vi "UpravljanjeHidraulicnomPumpom.vi"() -> ()   [LabVIEW 2014]
uses:
  Control 1.ctl
  <vilib>/functionblocks/Edge Detection/Edge Detect/Edge Detect.vi
  <vilib>/functionblocks/FB Core/FB Core.xnode
  <vilib>/functionblocks/NI_FunctionBlock Libraries.lvlib
panel:
  in  "stop":bool
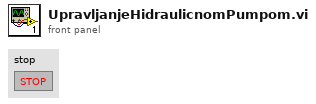
[diagram p1: front panel]
types:
  T1 = typedef "Control 1.ctl" = enum16{"System off", "System on", "Left", "Center", "Right", "Emergency off", ""}
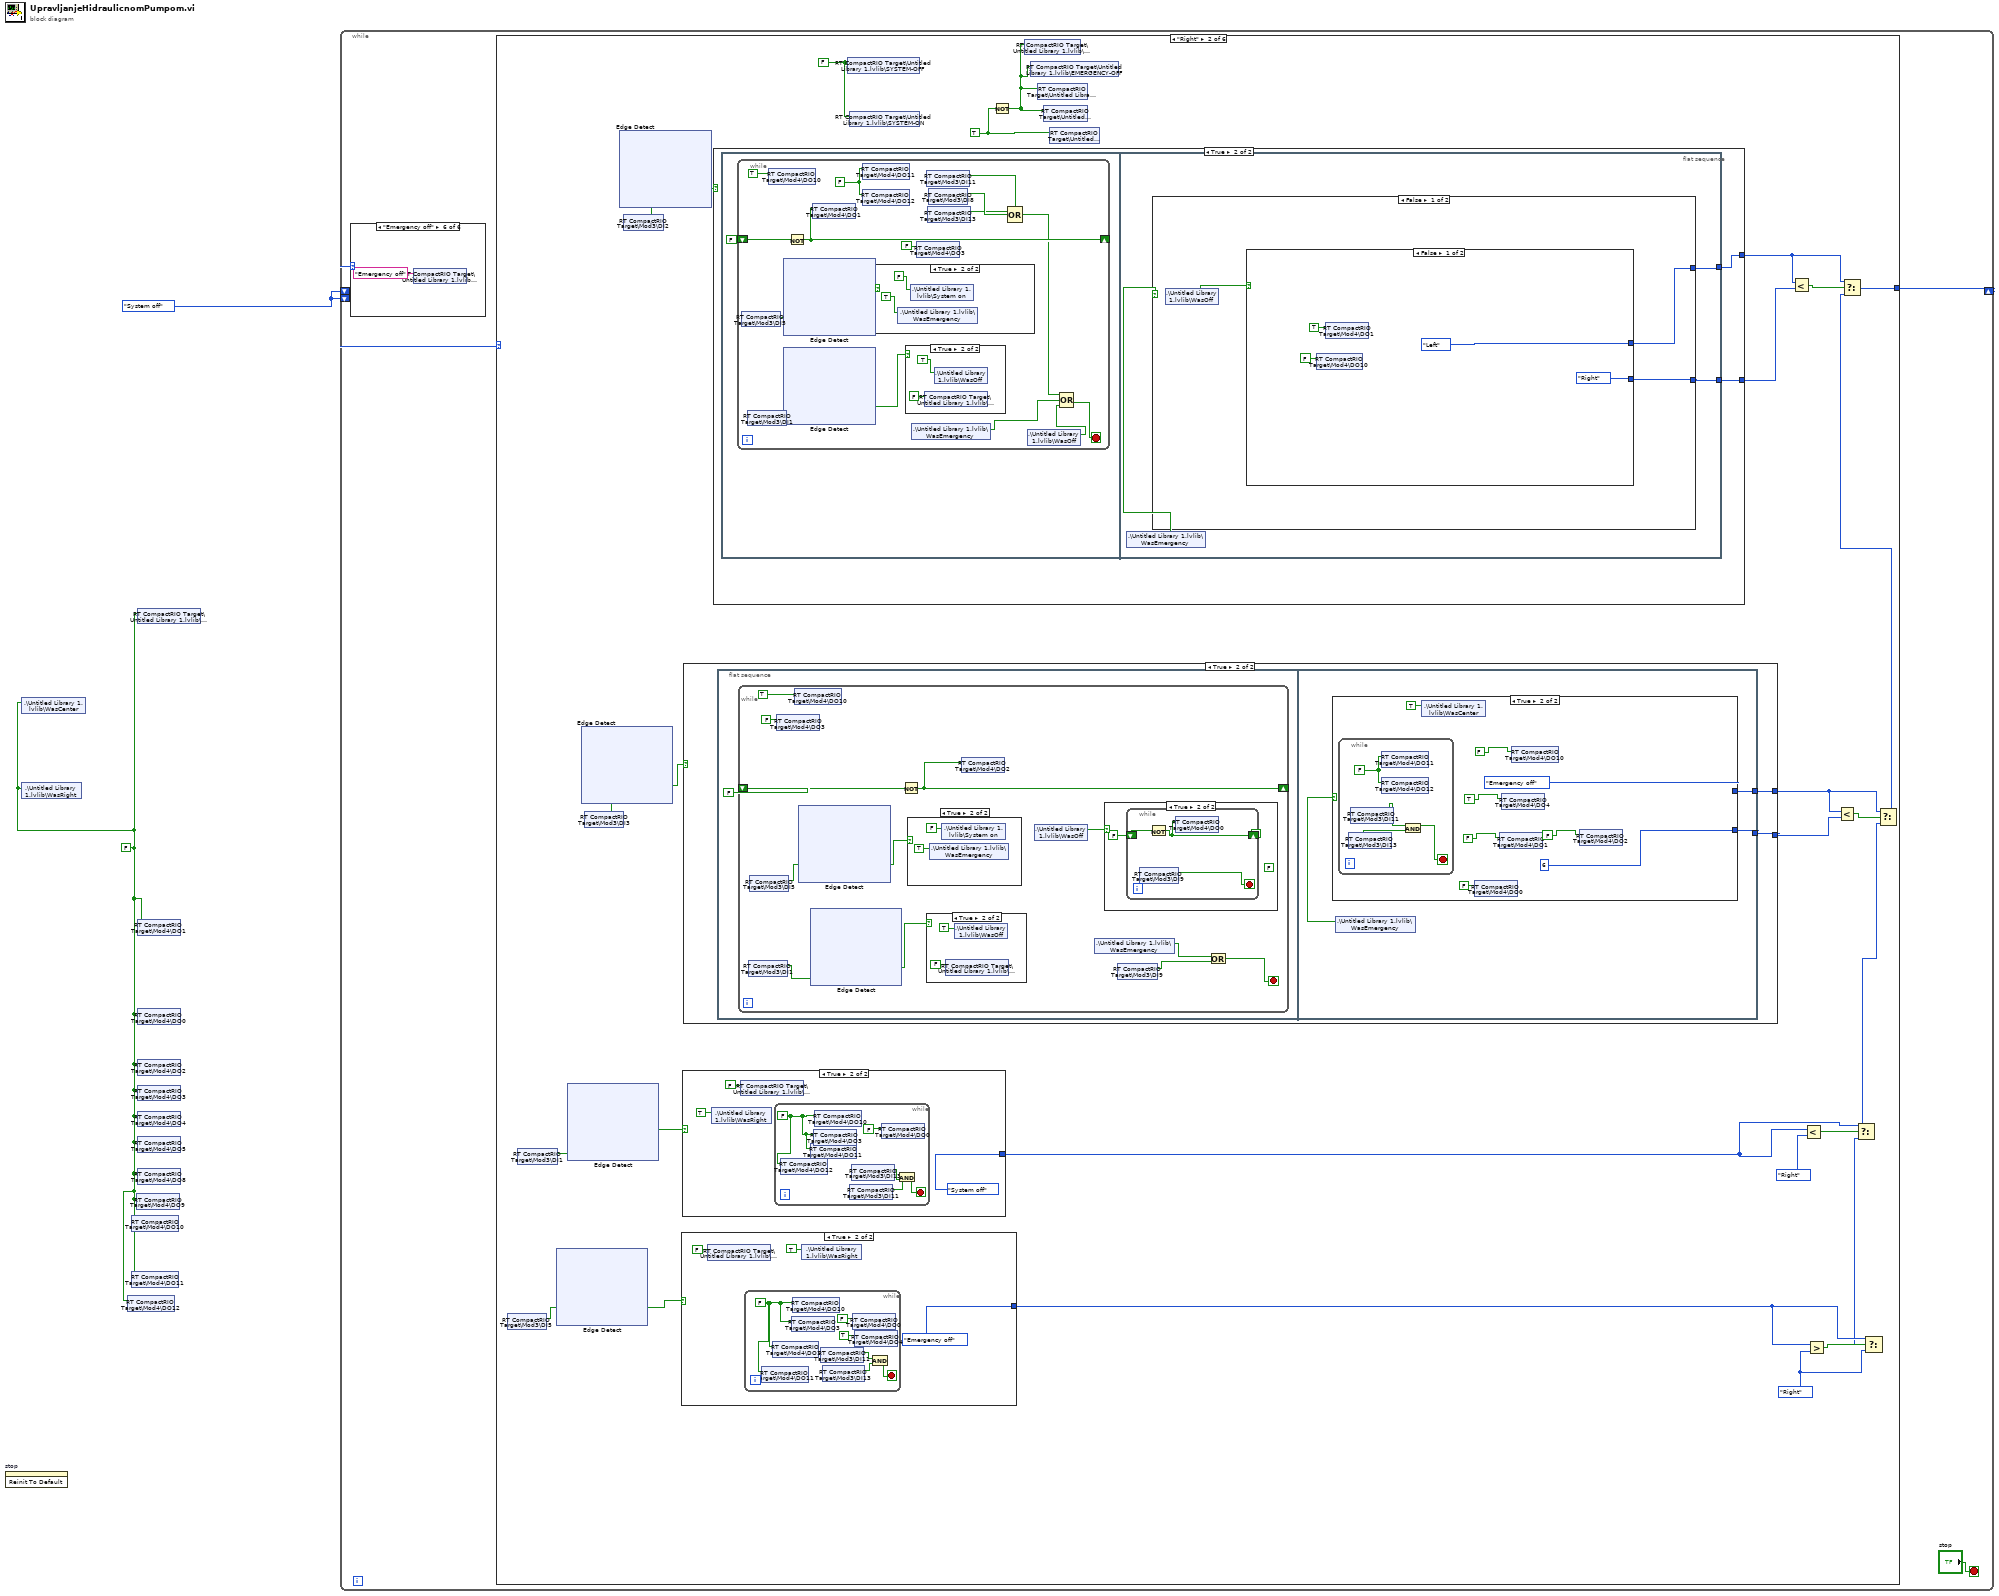
[diagram p0: block diagram]
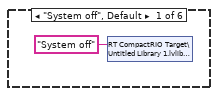
[diagram p2: hidden frame]
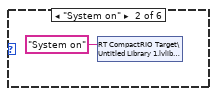
[diagram p3: hidden frame]
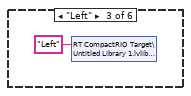
[diagram p4: hidden frame]
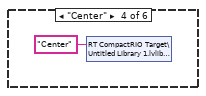
[diagram p5: hidden frame]
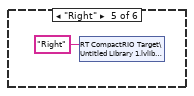
[diagram p6: hidden frame]
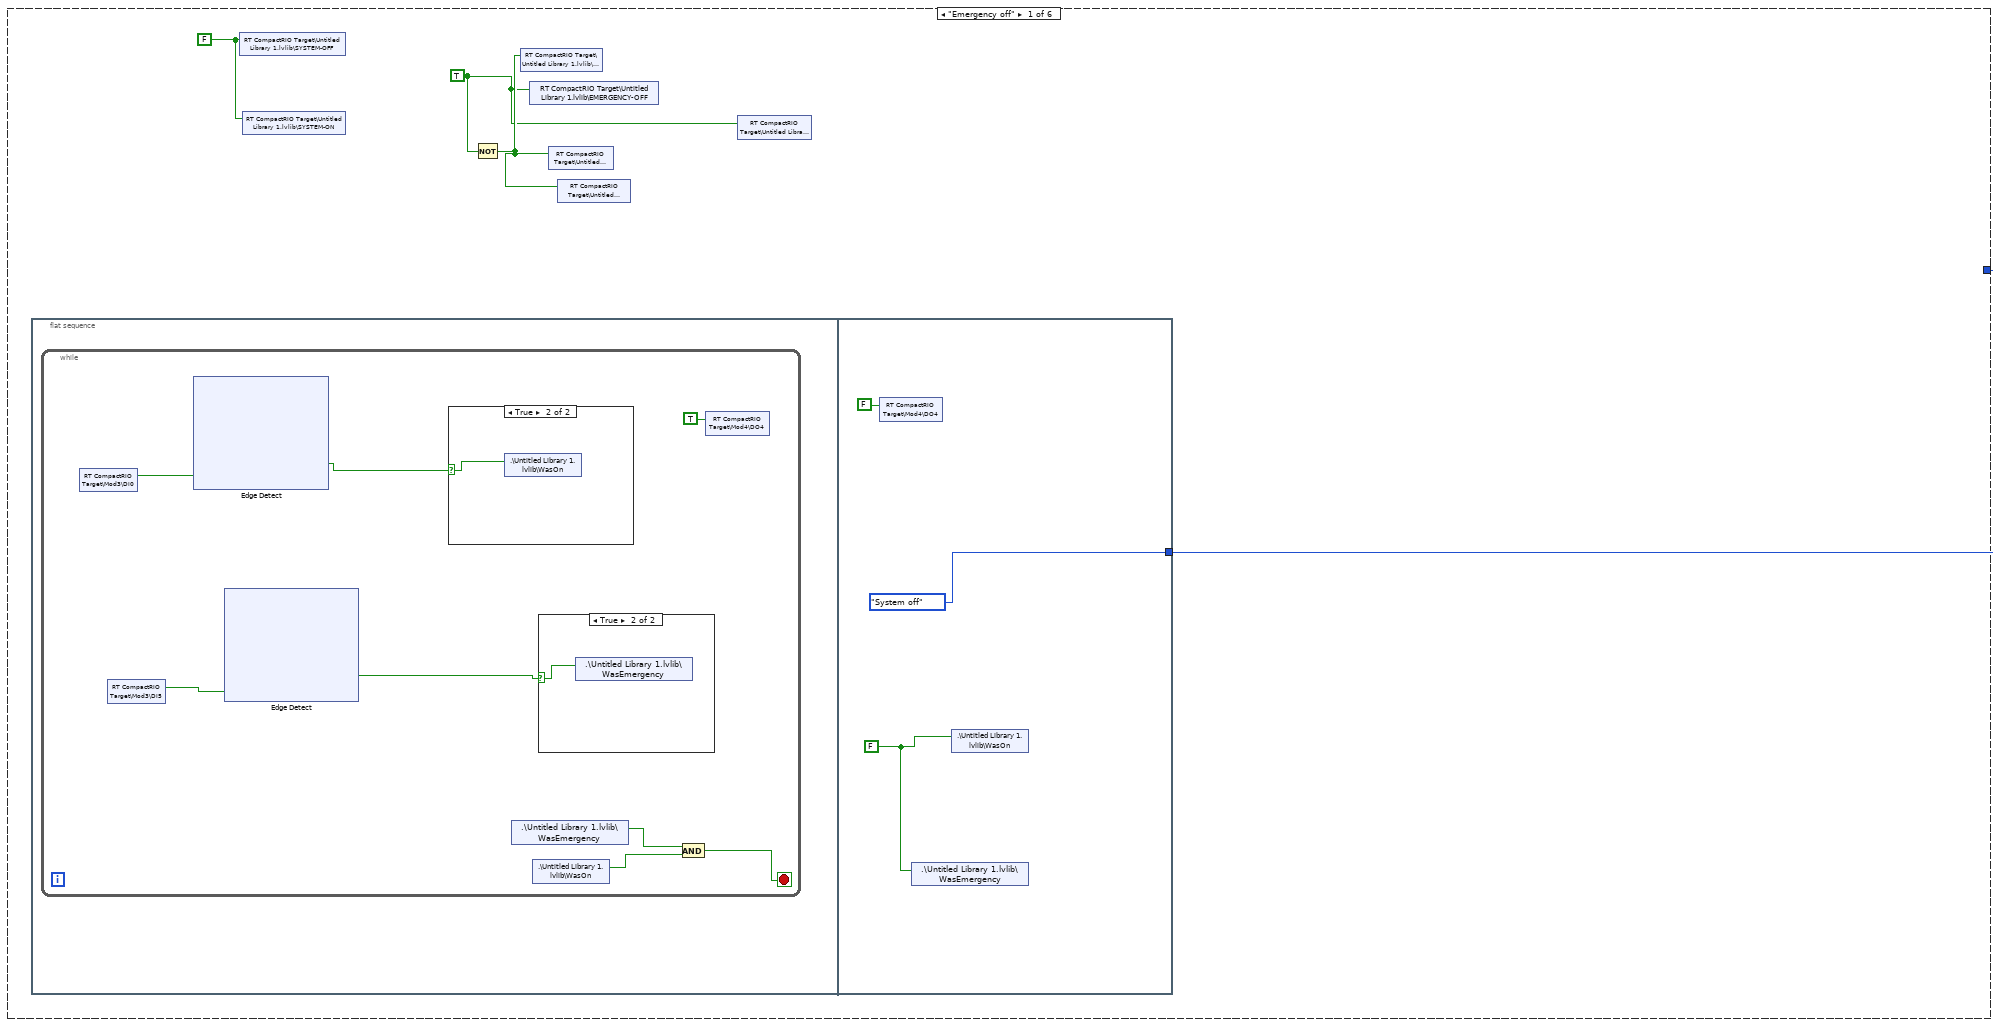
[diagram p7: hidden frame]
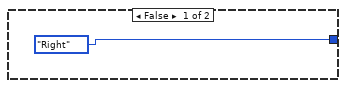
[diagram p10: hidden frame]
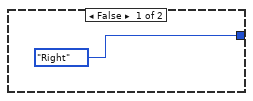
[diagram p11: hidden frame]
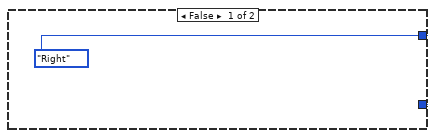
[diagram p12: hidden frame]
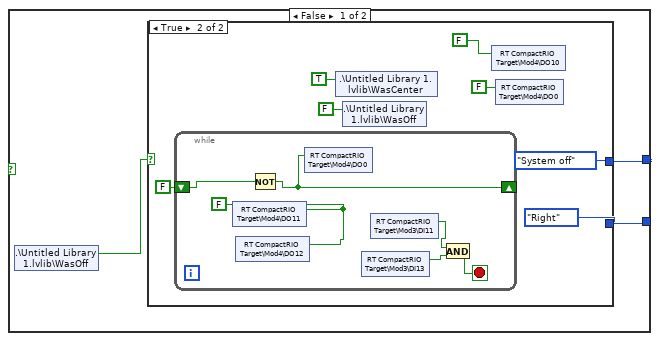
[diagram p16: hidden frame]
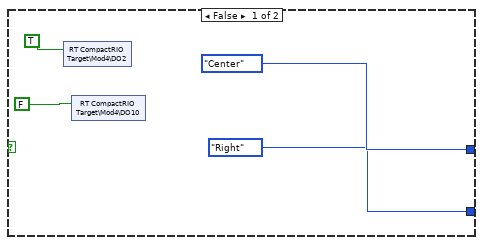
[diagram p17: hidden frame]
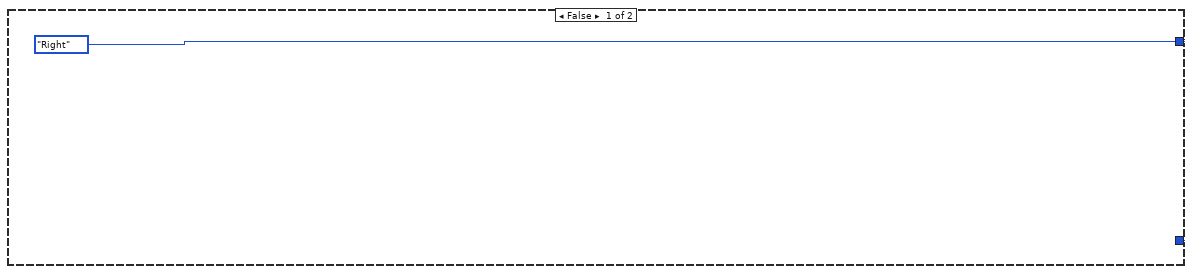
[diagram p18: hidden frame]
diagram:
  w2 = Control_1."System off" ("Enum")
  w1 = FALSE ("System on")
  n1 = invoke on="stop" class="Bool (strict)" method="Reinit To Default"() -> ()  [unwired: 3 in, 3 out]
  n2 = shared-variable ".\\Untitled Library 1.lvlib\\WasCenter"(w1) -> ()  [unwired: 1 in, 1 out]
  n3 = shared-variable ".\\Untitled Library 1.lvlib\\WasRight"(w1) -> ()  [unwired: 1 in, 1 out]
  n4 = shared-variable "RT CompactRIO Target\\Mod4\\DO12"(w1) -> ()  [unwired: 1 in, 1 out]
  n5 = shared-variable "RT CompactRIO Target\\Mod4\\DO10"(w1) -> ()  [unwired: 1 in, 1 out]
  n6 = shared-variable "RT CompactRIO Target\\Mod4\\DO11"(w1) -> ()  [unwired: 1 in, 1 out]
  n7 = shared-variable "RT CompactRIO Target\\Mod4\\DO9"(w1) -> ()  [unwired: 1 in, 1 out]
  n8 = shared-variable "RT CompactRIO Target\\Untitled Library 1.lvlib\\System on"(w1) -> ()  [unwired: 1 in, 1 out]
  n9 = shared-variable "RT CompactRIO Target\\Mod4\\DO1"(w1) -> ()  [unwired: 1 in, 1 out]
  n10 = shared-variable "RT CompactRIO Target\\Mod4\\DO0"(w1) -> ()  [unwired: 1 in, 1 out]
  n11 = shared-variable "RT CompactRIO Target\\Mod4\\DO2"(w1) -> ()  [unwired: 1 in, 1 out]
  n12 = shared-variable "RT CompactRIO Target\\Mod4\\DO3"(w1) -> ()  [unwired: 1 in, 1 out]
  n13 = shared-variable "RT CompactRIO Target\\Mod4\\DO4"(w1) -> ()  [unwired: 1 in, 1 out]
  n14 = shared-variable "RT CompactRIO Target\\Mod4\\DO5"(w1) -> ()  [unwired: 1 in, 1 out]
  n15 = shared-variable "RT CompactRIO Target\\Mod4\\DO8"(w1) -> ()  [unwired: 1 in, 1 out]
  n16 = while {
    shift-right: [w4] -> _
    shift-left: w2 -> [w3]
    shift-left: w2 -> [_]
    stop <- "stop" stop-if-true
    n17 = case shown="\"Emergency off\"" w3 {
      frame "System off", Default {
        n18 = shared-variable "RT CompactRIO Target\\Untitled Library 1.lvlib\\STANJE"("System off" ("STANJE")) -> ()  [unwired: 1 in, 1 out]
      }
      frame "System on" {
        n19 = shared-variable "RT CompactRIO Target\\Untitled Library 1.lvlib\\STANJE"("System on" ("STANJE")) -> ()  [unwired: 1 in, 1 out]
      }
      frame "Left" {
        n20 = shared-variable "RT CompactRIO Target\\Untitled Library 1.lvlib\\STANJE"("Left" ("STANJE")) -> ()  [unwired: 1 in, 1 out]
      }
      frame "Center" {
        n21 = shared-variable "RT CompactRIO Target\\Untitled Library 1.lvlib\\STANJE"("Center" ("STANJE")) -> ()  [unwired: 1 in, 1 out]
      }
      frame "Right" {
        n22 = shared-variable "RT CompactRIO Target\\Untitled Library 1.lvlib\\STANJE"("Right" ("STANJE")) -> ()  [unwired: 1 in, 1 out]
      }
      frame "Emergency off" {
        n23 = shared-variable "RT CompactRIO Target\\Untitled Library 1.lvlib\\STANJE"("Emergency off" ("STANJE")) -> ()  [unwired: 1 in, 1 out]
      }
    }
    n24 = case shown="\"Right\"" w3 {
      tunnel: [w15 w110 w592 w1059 w1532 w1594] -> w4
      frame "Emergency off" {
        w13 = FALSE ("SYSTEM-OFF")
        w12 = TRUE ("RIGHT")
        n25 = flat-sequence {
          tunnel: [Control_1."System off" ("Enum")] -> w15
          frame #0 {
            n26 = while {
              stop <- w21 stop-if-true
              n27 = shared-variable "RT CompactRIO Target\\Mod3\\DI0"() -> (w19:bool)  [unwired: 1 in, 1 out]
              n28 = shared-variable "RT CompactRIO Target\\Mod3\\DI5"() -> (w18:bool)  [unwired: 1 in, 1 out]
              n29 = xnode "Edge Detect"("input 1"=w19) -> ("output"=w17:bool)  [unwired: 2 in, 1 out]
              n30 = xnode "Edge Detect"("input 1"=w18) -> ("output"=w16:bool)  [unwired: 2 in, 1 out]
              n31 = case shown="True" w17 {
                selector: w17 -> [_ w25]
                frame False {
                }
                frame True {
                  n32 = shared-variable ".\\Untitled Library 1.lvlib\\WasOn"(w25) -> ()  [unwired: 1 in, 1 out]
                }
              }
              n33 = shared-variable ".\\Untitled Library 1.lvlib\\WasEmergency"() -> (w22:bool)  [unwired: 1 in, 1 out]
              n34 = shared-variable ".\\Untitled Library 1.lvlib\\WasOn"() -> (w23:bool)  [unwired: 1 in, 1 out]
              n35 = case shown="True" w16 {
                selector: w16 -> [_ w24]
                frame False {
                }
                frame True {
                  n36 = shared-variable ".\\Untitled Library 1.lvlib\\WasEmergency"(w24) -> ()  [unwired: 1 in, 1 out]
                }
              }
              n37 = And(x=w22, y=w23) -> (x .and. y?=w21:bool)
              n38 = shared-variable "RT CompactRIO Target\\Mod4\\DO4"(TRUE ("DO4")) -> ()  [unwired: 1 in, 1 out]
            }
          }
          frame #1 {
            w106 = FALSE ("WasOn")
            n39 = shared-variable "RT CompactRIO Target\\Mod4\\DO4"(FALSE ("DO4")) -> ()  [unwired: 1 in, 1 out]
            n40 = shared-variable ".\\Untitled Library 1.lvlib\\WasEmergency"(w106) -> ()  [unwired: 1 in, 1 out]
            n41 = shared-variable ".\\Untitled Library 1.lvlib\\WasOn"(w106) -> ()  [unwired: 1 in, 1 out]
          }
        }
        n42 = shared-variable "RT CompactRIO Target\\Untitled Library 1.lvlib\\SYSTEM-OFF"(w13) -> ()  [unwired: 1 in, 1 out]
        n43 = shared-variable "RT CompactRIO Target\\Untitled Library 1.lvlib\\SYSTEM-ON"(w13) -> ()  [unwired: 1 in, 1 out]
        n44 = Not(x=w12) -> (.not. x?=w14:bool)
        n45 = shared-variable "RT CompactRIO Target\\Untitled Library 1.lvlib\\CENTER"(w14) -> ()  [unwired: 1 in, 1 out]
        n46 = shared-variable "RT CompactRIO Target\\Untitled Library 1.lvlib\\EMERGENCY-OFF"(w12) -> ()  [unwired: 1 in, 1 out]
        n47 = shared-variable "RT CompactRIO Target\\Untitled Library 1.lvlib\\LEFT"(w14) -> ()  [unwired: 1 in, 1 out]
        n48 = shared-variable "RT CompactRIO Target\\Untitled Library 1.lvlib\\RIGHT"(w14) -> ()  [unwired: 1 in, 1 out]
        n49 = shared-variable "RT CompactRIO Target\\Untitled Library 1.lvlib\\FAULT"(w12) -> ()  [unwired: 1 in, 1 out]
      }
      frame "Right" {
        w109 = FALSE ("SYSTEM-OFF")
        w111 = Control_1."Right" ("y")
        w127 = TRUE ("RIGHT")
        n50 = shared-variable "RT CompactRIO Target\\Mod3\\DI5"() -> (w128:bool)  [unwired: 1 in, 1 out]
        n51 = shared-variable "RT CompactRIO Target\\Mod3\\DI1"() -> (w129:bool)  [unwired: 1 in, 1 out]
        n52 = xnode "Edge Detect"("input 2"=w128) -> ("output"=w130:bool)  [unwired: 2 in, 1 out]
        n53 = xnode "Edge Detect"("input 1"=w129) -> ("output"=w131:bool)  [unwired: 2 in, 1 out]
        n54 = shared-variable "RT CompactRIO Target\\Mod3\\DI3"() -> (w133:bool)  [unwired: 1 in, 1 out]
        n55 = xnode "Edge Detect"("input 1"=w133) -> ("output"=w132:bool)  [unwired: 2 in, 1 out]
        n56 = shared-variable "RT CompactRIO Target\\Mod3\\DI2"() -> (w135:bool)  [unwired: 1 in, 1 out]
        n57 = xnode "Edge Detect"("input 1"=w135) -> ("output"=w134:bool)  [unwired: 2 in, 1 out]
        n58 = case shown="True" w130 {
          tunnel: [Control_1."Right" ("Enum") Control_1."Emergency off" ("Enum")] -> w113
          frame False {
          }
          frame True {
            n59 = shared-variable "RT CompactRIO Target\\Untitled Library 1.lvlib\\System on"(FALSE ("System on")) -> ()  [unwired: 1 in, 1 out]
            n60 = while {
              stop <- w143 stop-if-true
              w142 = FALSE ("DO8")
              n61 = shared-variable "RT CompactRIO Target\\Mod4\\DO11"(w142) -> ()  [unwired: 1 in, 1 out]
              n62 = shared-variable "RT CompactRIO Target\\Mod4\\DO12"(w142) -> ()  [unwired: 1 in, 1 out]
              n63 = shared-variable "RT CompactRIO Target\\Mod4\\DO3"(w142) -> ()  [unwired: 1 in, 1 out]
              n64 = shared-variable "RT CompactRIO Target\\Mod4\\DO10"(w142) -> ()  [unwired: 1 in, 1 out]
              n65 = shared-variable "RT CompactRIO Target\\Mod3\\DI11"() -> (w144:bool)  [unwired: 1 in, 1 out]
              n66 = shared-variable "RT CompactRIO Target\\Mod3\\DI13"() -> (w145:bool)  [unwired: 1 in, 1 out]
              n67 = shared-variable "RT CompactRIO Target\\Mod4\\DO0"(FALSE ("DO4")) -> ()  [unwired: 1 in, 1 out]
              n68 = shared-variable "RT CompactRIO Target\\Mod4\\DO4"(TRUE ("DO4")) -> ()  [unwired: 1 in, 1 out]
              n69 = And(x=w144, y=w145) -> (x .and. y?=w143:bool)
            }
            n70 = shared-variable ".\\Untitled Library 1.lvlib\\WasRight"(TRUE ("WasCenter")) -> ()  [unwired: 1 in, 1 out]
          }
        }
        n71 = case shown="True" w131 {
          tunnel: [Control_1."Right" ("Enum") Control_1."System off" ("Enum")] -> w116
          frame False {
          }
          frame True {
            n72 = shared-variable ".\\Untitled Library 1.lvlib\\WasRight"(TRUE ("WasCenter")) -> ()  [unwired: 1 in, 1 out]
            n73 = shared-variable "RT CompactRIO Target\\Untitled Library 1.lvlib\\System on"(FALSE ("System on")) -> ()  [unwired: 1 in, 1 out]
            n74 = while {
              stop <- w192 stop-if-true
              w191 = FALSE ("DO8")
              n75 = shared-variable "RT CompactRIO Target\\Mod4\\DO12"(w191) -> ()  [unwired: 1 in, 1 out]
              n76 = shared-variable "RT CompactRIO Target\\Mod4\\DO11"(w191) -> ()  [unwired: 1 in, 1 out]
              n77 = shared-variable "RT CompactRIO Target\\Mod4\\DO3"(w191) -> ()  [unwired: 1 in, 1 out]
              n78 = shared-variable "RT CompactRIO Target\\Mod4\\DO10"(w191) -> ()  [unwired: 1 in, 1 out]
              n79 = shared-variable "RT CompactRIO Target\\Mod3\\DI11"() -> (w193:bool)  [unwired: 1 in, 1 out]
              n80 = shared-variable "RT CompactRIO Target\\Mod3\\DI13"() -> (w194:bool)  [unwired: 1 in, 1 out]
              n81 = shared-variable "RT CompactRIO Target\\Mod4\\DO0"(FALSE ("DO8")) -> ()  [unwired: 1 in, 1 out]
              n82 = And(x=w193, y=w194) -> (x .and. y?=w192:bool)
            }
          }
        }
        n83 = case shown="True" w132 {
          tunnel: [w235 w237] -> w120
          tunnel: [w235 w236] -> w122
          frame False {
            w235 = Control_1."Right" ("Enum")
          }
          frame True {
            n84 = flat-sequence {
              tunnel: [w340] -> w237
              tunnel: [w339] -> w236
              frame #0 {
                n85 = while {
                  shift-right: [w249] -> _
                  shift-left: FALSE ("DO8") -> [w250]
                  stop <- w242 stop-if-true
                  n86 = shared-variable "RT CompactRIO Target\\Mod3\\DI1"() -> (w240:bool)  [unwired: 1 in, 1 out]
                  n87 = shared-variable "RT CompactRIO Target\\Mod3\\DI5"() -> (w246:bool)  [unwired: 1 in, 1 out]
                  n88 = shared-variable "RT CompactRIO Target\\Mod4\\DO3"(FALSE ("DO3")) -> ()  [unwired: 1 in, 1 out]
                  n89 = shared-variable "RT CompactRIO Target\\Mod4\\DO10"(TRUE ("DO8")) -> ()  [unwired: 1 in, 1 out]
                  n90 = xnode "Edge Detect"("input 2"=w246) -> ("output"=w245:bool)  [unwired: 2 in, 1 out]
                  n91 = xnode "Edge Detect"("input 1"=w240) -> ("output"=w239:bool)  [unwired: 2 in, 1 out]
                  n92 = Not(x=w250) -> (.not. x?=w249:bool)
                  n93 = case shown="True" w245 {
                    frame False {
                    }
                    frame True {
                      n94 = shared-variable ".\\Untitled Library 1.lvlib\\WasEmergency"(TRUE ("WasEmergency")) -> ()  [unwired: 1 in, 1 out]
                      n95 = shared-variable ".\\Untitled Library 1.lvlib\\System on"(FALSE ("System on")) -> ()  [unwired: 1 in, 1 out]
                    }
                  }
                  n96 = case shown="True" w239 {
                    frame False {
                    }
                    frame True {
                      n97 = shared-variable "RT CompactRIO Target\\Untitled Library 1.lvlib\\System on"(FALSE ("System on")) -> ()  [unwired: 1 in, 1 out]
                      n98 = shared-variable ".\\Untitled Library 1.lvlib\\WasOff"(TRUE ("WasOff")) -> ()  [unwired: 1 in, 1 out]
                    }
                  }
                  n99 = shared-variable "RT CompactRIO Target\\Mod4\\DO2"(w249) -> ()  [unwired: 1 in, 1 out]
                  n100 = shared-variable ".\\Untitled Library 1.lvlib\\WasOff"() -> (w241:bool)  [unwired: 1 in, 1 out]
                  n101 = shared-variable ".\\Untitled Library 1.lvlib\\WasEmergency"() -> (w244:bool)  [unwired: 1 in, 1 out]
                  n102 = case shown="True" w241 {
                    frame False {
                    }
                    frame True {
                      (unwired) FALSE ("WasOff")
                      (unwired) FALSE ("DO8")
                      n103 = while {
                        shift-right: [w252] -> _
                        shift-left: FALSE -> [w254]
                        stop <- w253 stop-if-true
                        n104 = shared-variable "RT CompactRIO Target\\Mod3\\DI9"() -> (w253:bool)  [unwired: 1 in, 1 out]
                        n105 = Not(x=w254) -> (.not. x?=w252:bool)
                        n106 = shared-variable "RT CompactRIO Target\\Mod4\\DO0"(w252) -> ()  [unwired: 1 in, 1 out]
                      }
                    }
                  }
                  n107 = shared-variable "RT CompactRIO Target\\Mod3\\DI9"() -> (w243:bool)  [unwired: 1 in, 1 out]
                  n108 = Or(x=w244, y=w243) -> (x .or. y?=w242:bool)
                }
              }
              frame #1 {
                n109 = shared-variable ".\\Untitled Library 1.lvlib\\WasEmergency"() -> (w341:bool)  [unwired: 1 in, 1 out]
                n110 = case shown="True" w341 {
                  tunnel: [w343 Control_1."Emergency off" ("Enum")] -> w340
                  tunnel: [w342 6] -> w339
                  frame False {
                    n111 = shared-variable ".\\Untitled Library 1.lvlib\\WasOff"() -> (w344:bool)  [unwired: 1 in, 1 out]
                    n112 = case shown="True" w344 {
                      tunnel: [Control_1."Center" ("Enum") Control_1."System off" ("Enum")] -> w343
                      tunnel: [Control_1."Right" ("Enum") Control_1."Right" ("Enum")] -> w342
                      frame False {
                        n113 = shared-variable "RT CompactRIO Target\\Mod4\\DO2"(TRUE ("DO12")) -> ()  [unwired: 1 in, 1 out]
                        n114 = shared-variable "RT CompactRIO Target\\Mod4\\DO10"(FALSE ("DO8")) -> ()  [unwired: 1 in, 1 out]
                      }
                      frame True {
                        n115 = while {
                          shift-right: [w356] -> _
                          shift-left: FALSE -> [w357]
                          stop <- w358 stop-if-true
                          w361 = FALSE ("DO11")
                          n116 = shared-variable "RT CompactRIO Target\\Mod4\\DO11"(w361) -> ()  [unwired: 1 in, 1 out]
                          n117 = shared-variable "RT CompactRIO Target\\Mod4\\DO12"(w361) -> ()  [unwired: 1 in, 1 out]
                          n118 = Not(x=w357) -> (.not. x?=w356:bool)
                          n119 = shared-variable "RT CompactRIO Target\\Mod4\\DO0"(w356) -> ()  [unwired: 1 in, 1 out]
                          n120 = shared-variable "RT CompactRIO Target\\Mod3\\DI13"() -> (w359:bool)  [unwired: 1 in, 1 out]
                          n121 = shared-variable "RT CompactRIO Target\\Mod3\\DI11"() -> (w360:bool)  [unwired: 1 in, 1 out]
                          n122 = And(x=w360, y=w359) -> (x .and. y?=w358:bool)
                        }
                        n123 = shared-variable ".\\Untitled Library 1.lvlib\\WasCenter"(TRUE ("WasRight")) -> ()  [unwired: 1 in, 1 out]
                        n124 = shared-variable ".\\Untitled Library 1.lvlib\\WasOff"(FALSE ("WasOff")) -> ()  [unwired: 1 in, 1 out]
                        n125 = shared-variable "RT CompactRIO Target\\Mod4\\DO10"(FALSE ("DO0")) -> ()  [unwired: 1 in, 1 out]
                        n126 = shared-variable "RT CompactRIO Target\\Mod4\\DO0"(FALSE ("DO0")) -> ()  [unwired: 1 in, 1 out]
                      }
                    }
                  }
                  frame True {
                    n127 = while {
                      stop <- w370 stop-if-true
                      w373 = FALSE ("DO8")
                      n128 = shared-variable "RT CompactRIO Target\\Mod3\\DI13"() -> (w371:bool)  [unwired: 1 in, 1 out]
                      n129 = shared-variable "RT CompactRIO Target\\Mod3\\DI11"() -> (w372:bool)  [unwired: 1 in, 1 out]
                      n130 = shared-variable "RT CompactRIO Target\\Mod4\\DO11"(w373) -> ()  [unwired: 1 in, 1 out]
                      n131 = shared-variable "RT CompactRIO Target\\Mod4\\DO12"(w373) -> ()  [unwired: 1 in, 1 out]
                      n132 = And(x=w372, y=w371) -> (x .and. y?=w370:bool)
                    }
                    n133 = shared-variable ".\\Untitled Library 1.lvlib\\WasCenter"(TRUE ("WasRight")) -> ()  [unwired: 1 in, 1 out]
                    n134 = shared-variable "RT CompactRIO Target\\Mod4\\DO0"(FALSE ("DO0")) -> ()  [unwired: 1 in, 1 out]
                    n135 = shared-variable "RT CompactRIO Target\\Mod4\\DO1"(FALSE ("DO8")) -> ()  [unwired: 1 in, 1 out]
                    n136 = shared-variable "RT CompactRIO Target\\Mod4\\DO4"(TRUE ("DO8")) -> ()  [unwired: 1 in, 1 out]
                    n137 = shared-variable "RT CompactRIO Target\\Mod4\\DO10"(FALSE ("DO8")) -> ()  [unwired: 1 in, 1 out]
                    n138 = shared-variable "RT CompactRIO Target\\Mod4\\DO2"(FALSE ("DO8")) -> ()  [unwired: 1 in, 1 out]
                  }
                }
              }
            }
          }
        }
        n139 = case shown="True" w134 {
          tunnel: [w414 w416] -> w123
          tunnel: [w414 w415] -> w125
          frame False {
            w414 = Control_1."Right" ("Enum")
          }
          frame True {
            n140 = flat-sequence {
              tunnel: [w519] -> w416
              tunnel: [w518] -> w415
              frame #0 {
                n141 = while {
                  shift-right: [w431] -> _
                  shift-left: FALSE ("DO8") -> [w432]
                  stop <- w420 stop-if-true
                  w427 = FALSE ("DO8")
                  n142 = shared-variable "RT CompactRIO Target\\Mod3\\DI5"() -> (w424:bool)  [unwired: 1 in, 1 out]
                  n143 = shared-variable "RT CompactRIO Target\\Mod3\\DI1"() -> (w425:bool)  [unwired: 1 in, 1 out]
                  n144 = shared-variable "RT CompactRIO Target\\Mod4\\DO10"(TRUE ("DO8")) -> ()  [unwired: 1 in, 1 out]
                  n145 = xnode "Edge Detect"("input 2"=w424) -> ("output"=w423:bool)  [unwired: 2 in, 1 out]
                  n146 = xnode "Edge Detect"("input 1"=w425) -> ("output"=w419:bool)  [unwired: 2 in, 1 out]
                  n147 = Not(x=w432) -> (.not. x?=w431:bool)
                  n148 = shared-variable "RT CompactRIO Target\\Mod4\\DO1"(w431) -> ()  [unwired: 1 in, 1 out]
                  n149 = shared-variable "RT CompactRIO Target\\Mod4\\DO11"(w427) -> ()  [unwired: 1 in, 1 out]
                  n150 = shared-variable "RT CompactRIO Target\\Mod4\\DO12"(w427) -> ()  [unwired: 1 in, 1 out]
                  n151 = case shown="True" w423 {
                    frame False {
                    }
                    frame True {
                      n152 = shared-variable ".\\Untitled Library 1.lvlib\\WasEmergency"(TRUE ("WasEmergency")) -> ()  [unwired: 1 in, 1 out]
                      n153 = shared-variable ".\\Untitled Library 1.lvlib\\System on"(FALSE ("System on")) -> ()  [unwired: 1 in, 1 out]
                    }
                  }
                  n154 = case shown="True" w419 {
                    frame False {
                    }
                    frame True {
                      n155 = shared-variable "RT CompactRIO Target\\Untitled Library 1.lvlib\\System on"(FALSE ("System on")) -> ()  [unwired: 1 in, 1 out]
                      n156 = shared-variable ".\\Untitled Library 1.lvlib\\WasOff"(TRUE ("WasOff")) -> ()  [unwired: 1 in, 1 out]
                    }
                  }
                  n157 = shared-variable ".\\Untitled Library 1.lvlib\\WasEmergency"() -> (w421:bool)  [unwired: 1 in, 1 out]
                  n158 = shared-variable "RT CompactRIO Target\\Mod4\\DO3"(FALSE ("DO3")) -> ()  [unwired: 1 in, 1 out]
                  n159 = shared-variable "RT CompactRIO Target\\Mod3\\DI11"() -> (w430:bool)  [unwired: 1 in, 1 out]
                  n160 = shared-variable "RT CompactRIO Target\\Mod3\\DI13"() -> (w428:bool)  [unwired: 1 in, 1 out]
                  n161 = shared-variable "RT CompactRIO Target\\Mod3\\DI8"() -> (w429:bool)  [unwired: 1 in, 1 out]
                  n162 = Compound Arithmetic op=OR(w430, w429, w428) -> (w418:bool)
                  n163 = shared-variable ".\\Untitled Library 1.lvlib\\WasOff"() -> (w422:bool)  [unwired: 1 in, 1 out]
                  n164 = Compound Arithmetic op=OR(w418, w421, w422) -> (w420:bool)
                }
              }
              frame #1 {
                n165 = shared-variable ".\\Untitled Library 1.lvlib\\WasEmergency"() -> (w520:bool)  [unwired: 1 in, 1 out]
                n166 = case shown="False" w520 {
                  tunnel: [w522 Control_1."Emergency off" ("Enum")] -> w519
                  tunnel: [w521 6] -> w518
                  frame False {
                    n167 = shared-variable ".\\Untitled Library 1.lvlib\\WasOff"() -> (w523:bool)  [unwired: 1 in, 1 out]
                    n168 = case shown="False" w523 {
                      tunnel: [Control_1."Left" ("Enum") Control_1."System off" ("Enum")] -> w522
                      tunnel: [Control_1."Right" ("Enum") Control_1."Right" ("Enum")] -> w521
                      frame False {
                        n169 = shared-variable "RT CompactRIO Target\\Mod4\\DO10"(FALSE ("DO1")) -> ()  [unwired: 1 in, 1 out]
                        n170 = shared-variable "RT CompactRIO Target\\Mod4\\DO1"(TRUE ("DO3")) -> ()  [unwired: 1 in, 1 out]
                      }
                      frame True {
                        n171 = flat-sequence {
                          frame #0 {
                            n172 = while {
                              shift-right: [w538] -> _
                              shift-left: FALSE -> [w539]
                              stop <- w534 stop-if-true
                              w537 = FALSE ("DO8")
                              n173 = shared-variable "RT CompactRIO Target\\Mod4\\DO10"(TRUE ("DO1")) -> ()  [unwired: 1 in, 1 out]
                              n174 = shared-variable "RT CompactRIO Target\\Mod3\\DI13"() -> (w535:bool)  [unwired: 1 in, 1 out]
                              n175 = shared-variable "RT CompactRIO Target\\Mod3\\DI11"() -> (w536:bool)  [unwired: 1 in, 1 out]
                              n176 = shared-variable "RT CompactRIO Target\\Mod3\\DI8"() -> (w532:bool)  [unwired: 1 in, 1 out]
                              n177 = Not(x=w539) -> (.not. x?=w538:bool)
                              n178 = Compound Arithmetic op=AND(w536, w535, w532) -> (w534:bool)
                              n179 = shared-variable "RT CompactRIO Target\\Mod4\\DO11"(w537) -> ()  [unwired: 1 in, 1 out]
                              n180 = shared-variable "RT CompactRIO Target\\Mod4\\DO12"(w537) -> ()  [unwired: 1 in, 1 out]
                              n181 = shared-variable "RT CompactRIO Target\\Mod4\\DO0"(w538) -> ()  [unwired: 1 in, 1 out]
                            }
                          }
                          frame #1 {
                            n182 = shared-variable "RT CompactRIO Target\\Mod4\\DO10"(FALSE ("DO1")) -> ()  [unwired: 1 in, 1 out]
                          }
                        }
                        n183 = shared-variable ".\\Untitled Library 1.lvlib\\WasOff"(FALSE ("WasOff")) -> ()  [unwired: 1 in, 1 out]
                      }
                    }
                  }
                  frame True {
                    n184 = while {
                      stop <- w548 stop-if-true
                      w551 = FALSE ("DO8")
                      n185 = shared-variable "RT CompactRIO Target\\Mod3\\DI13"() -> (w549:bool)  [unwired: 1 in, 1 out]
                      n186 = shared-variable "RT CompactRIO Target\\Mod3\\DI11"() -> (w550:bool)  [unwired: 1 in, 1 out]
                      n187 = And(x=w550, y=w549) -> (x .and. y?=w548:bool)
                      n188 = shared-variable "RT CompactRIO Target\\Mod4\\DO11"(w551) -> ()  [unwired: 1 in, 1 out]
                      n189 = shared-variable "RT CompactRIO Target\\Mod4\\DO12"(w551) -> ()  [unwired: 1 in, 1 out]
                    }
                    n190 = shared-variable ".\\Untitled Library 1.lvlib\\WasRight"(TRUE ("WasRight")) -> ()  [unwired: 1 in, 1 out]
                    n191 = shared-variable "RT CompactRIO Target\\Mod4\\DO1"(FALSE ("DO8")) -> ()  [unwired: 1 in, 1 out]
                    n192 = shared-variable "RT CompactRIO Target\\Mod4\\DO4"(TRUE ("DO8")) -> ()  [unwired: 1 in, 1 out]
                    n193 = shared-variable "RT CompactRIO Target\\Mod4\\DO10"(FALSE ("DO8")) -> ()  [unwired: 1 in, 1 out]
                    n194 = shared-variable "RT CompactRIO Target\\Mod4\\DO0"(FALSE ("DO0")) -> ()  [unwired: 1 in, 1 out]
                  }
                }
              }
            }
          }
        }
        n195 = shared-variable "RT CompactRIO Target\\Untitled Library 1.lvlib\\SYSTEM-OFF"(w109) -> ()  [unwired: 1 in, 1 out]
        n196 = shared-variable "RT CompactRIO Target\\Untitled Library 1.lvlib\\SYSTEM-ON"(w109) -> ()  [unwired: 1 in, 1 out]
        n197 = Not(x=w127) -> (.not. x?=w126:bool)
        n198 = shared-variable "RT CompactRIO Target\\Untitled Library 1.lvlib\\CENTER"(w126) -> ()  [unwired: 1 in, 1 out]
        n199 = shared-variable "RT CompactRIO Target\\Untitled Library 1.lvlib\\EMERGENCY-OFF"(w126) -> ()  [unwired: 1 in, 1 out]
        n200 = shared-variable "RT CompactRIO Target\\Untitled Library 1.lvlib\\FAULT"(w126) -> ()  [unwired: 1 in, 1 out]
        n201 = shared-variable "RT CompactRIO Target\\Untitled Library 1.lvlib\\LEFT"(w126) -> ()  [unwired: 1 in, 1 out]
        n202 = shared-variable "RT CompactRIO Target\\Untitled Library 1.lvlib\\RIGHT"(w127) -> ()  [unwired: 1 in, 1 out]
        n203 = Less?(x=w123, y=w125) -> (x < y?=w124:bool)
        n204 = Less?(x=w116, y=Control_1."Right") -> (x < y?=w117:bool)
        n205 = Greater?(x=w113, y=w111) -> (0:w114:bool)
        n206 = Less?(x=w120, y=w122) -> (x < y?=w121:bool)
        n207 = Select(t=w113, s=w114, f=w111) -> (s? t:f=w112:T1)
        n208 = Select(t=w116, s=w117, f=w112) -> (s? t:f=w115:T1)
        n209 = Select(t=w120, s=w121, f=w115) -> (s? t:f=w119:T1)
        n210 = Select(t=w123, s=w124, f=w119) -> (s? t:f=w110:T1)
      }
      frame "Center" {
        w594 = Control_1."Center" ("y")
        w612 = FALSE ("SYSTEM-OFF")
        w614 = TRUE ("RIGHT")
        n211 = shared-variable "RT CompactRIO Target\\Mod3\\DI4"() -> (w607:bool)  [unwired: 1 in, 1 out]
        n212 = shared-variable "RT CompactRIO Target\\Mod3\\DI5"() -> (w615:bool)  [unwired: 1 in, 1 out]
        n213 = xnode "Edge Detect"("input 1"=w607) -> ("output"=w606:bool)  [unwired: 2 in, 1 out]
        n214 = shared-variable "RT CompactRIO Target\\Mod3\\DI1"() -> (w618:bool)  [unwired: 1 in, 1 out]
        n215 = xnode "Edge Detect"("input 2"=w615) -> ("output"=w616:bool)  [unwired: 2 in, 1 out]
        n216 = shared-variable "RT CompactRIO Target\\Mod3\\DI2"() -> (w593:bool)  [unwired: 1 in, 1 out]
        n217 = xnode "Edge Detect"("input 1"=w593) -> ("output"=w611:bool)  [unwired: 2 in, 1 out]
        n218 = xnode "Edge Detect"("input 1"=w618) -> ("output"=w617:bool)  [unwired: 2 in, 1 out]
        n219 = shared-variable "RT CompactRIO Target\\Untitled Library 1.lvlib\\SYSTEM-OFF"(w612) -> ()  [unwired: 1 in, 1 out]
        n220 = shared-variable "RT CompactRIO Target\\Untitled Library 1.lvlib\\SYSTEM-ON"(w612) -> ()  [unwired: 1 in, 1 out]
        n221 = case shown="True" w606 {
          tunnel: [w710 w712] -> w603
          tunnel: [w710 w711] -> w605
          frame False {
            w710 = Control_1."Center" ("Enum")
          }
          frame True {
            n222 = flat-sequence {
              tunnel: [w818] -> w712
              tunnel: [w817] -> w711
              frame #0 {
                n223 = while {
                  shift-right: [w727] -> _
                  shift-left: FALSE ("DO8") -> [w728]
                  stop <- w714 stop-if-true
                  w726 = TRUE ("DO8")
                  n224 = shared-variable "RT CompactRIO Target\\Mod3\\DI1"() -> (w724:bool)  [unwired: 1 in, 1 out]
                  n225 = shared-variable "RT CompactRIO Target\\Mod3\\DI5"() -> (w723:bool)  [unwired: 1 in, 1 out]
                  n226 = shared-variable "RT CompactRIO Target\\Mod4\\DO9"(w726) -> ()  [unwired: 1 in, 1 out]
                  n227 = shared-variable "RT CompactRIO Target\\Mod4\\DO11"(w726) -> ()  [unwired: 1 in, 1 out]
                  n228 = shared-variable "RT CompactRIO Target\\Mod4\\DO12"(w726) -> ()  [unwired: 1 in, 1 out]
                  n229 = xnode "Edge Detect"("input 2"=w723) -> ("output"=w722:bool)  [unwired: 2 in, 1 out]
                  n230 = xnode "Edge Detect"("input 1"=w724) -> ("output"=w717:bool)  [unwired: 2 in, 1 out]
                  n231 = shared-variable "RT CompactRIO Target\\Mod4\\DO2"(FALSE ("DO2")) -> ()  [unwired: 1 in, 1 out]
                  n232 = Not(x=w728) -> (.not. x?=w727:bool)
                  n233 = shared-variable "RT CompactRIO Target\\Mod4\\DO3"(w727) -> ()  [unwired: 1 in, 1 out]
                  n234 = case shown="True" w722 {
                    frame False {
                    }
                    frame True {
                      n235 = shared-variable ".\\Untitled Library 1.lvlib\\WasEmergency"(TRUE ("WasEmergency")) -> ()  [unwired: 1 in, 1 out]
                      n236 = shared-variable ".\\Untitled Library 1.lvlib\\System on"(FALSE ("System on")) -> ()  [unwired: 1 in, 1 out]
                    }
                  }
                  n237 = case shown="True" w717 {
                    frame False {
                    }
                    frame True {
                      n238 = shared-variable "RT CompactRIO Target\\Untitled Library 1.lvlib\\System on"(FALSE ("System on")) -> ()  [unwired: 1 in, 1 out]
                      n239 = shared-variable ".\\Untitled Library 1.lvlib\\WasOff"(TRUE ("WasOff")) -> ()  [unwired: 1 in, 1 out]
                    }
                  }
                  n240 = shared-variable ".\\Untitled Library 1.lvlib\\WasOff"() -> (w716:bool)  [unwired: 1 in, 1 out]
                  n241 = shared-variable "RT CompactRIO Target\\Mod3\\DI12"() -> (w720:bool)  [unwired: 1 in, 1 out]
                  n242 = shared-variable "RT CompactRIO Target\\Mod3\\DI14"() -> (w719:bool)  [unwired: 1 in, 1 out]
                  n243 = shared-variable "RT CompactRIO Target\\Mod3\\DI10"() -> (w721:bool)  [unwired: 1 in, 1 out]
                  n244 = case shown="True" w716 {
                    frame False {
                    }
                    frame True {
                      (unwired) FALSE ("WasOff")
                      (unwired) FALSE ("DO8")
                      n245 = while {
                        shift-right: [w730] -> _
                        shift-left: FALSE -> [w732]
                        stop <- w731 stop-if-true
                        n246 = shared-variable "RT CompactRIO Target\\Mod3\\DI12"() -> (w731:bool)  [unwired: 1 in, 1 out]
                        n247 = Not(x=w732) -> (.not. x?=w730:bool)
                        n248 = shared-variable "RT CompactRIO Target\\Mod4\\DO0"(w730) -> ()  [unwired: 1 in, 1 out]
                      }
                    }
                  }
                  n249 = Compound Arithmetic op=AND(w721, w720, w719) -> (w718:bool)
                  n250 = shared-variable ".\\Untitled Library 1.lvlib\\WasEmergency"() -> (w715:bool)  [unwired: 1 in, 1 out]
                  n251 = Or(x=w715, y=w718) -> (x .or. y?=w714:bool)
                }
              }
              frame #1 {
                n252 = shared-variable ".\\Untitled Library 1.lvlib\\WasEmergency"() -> (w819:bool)  [unwired: 1 in, 1 out]
                n253 = case shown="True" w819 {
                  tunnel: [w820 Control_1."Emergency off" ("Enum")] -> w818
                  tunnel: [w821 Control_1."Center" ("Enum")] -> w817
                  frame False {
                    n254 = shared-variable ".\\Untitled Library 1.lvlib\\WasOff"() -> (w822:bool)  [unwired: 1 in, 1 out]
                    n255 = case shown="True" w822 {
                      tunnel: [Control_1."Center" ("Enum") -1] -> w821
                      tunnel: [Control_1."Right" ("Enum") Control_1."System off" ("Enum")] -> w820
                      frame False {
                        n256 = shared-variable "RT CompactRIO Target\\Mod4\\DO9"(FALSE ("DO8")) -> ()  [unwired: 1 in, 1 out]
                        n257 = shared-variable "RT CompactRIO Target\\Mod4\\DO3"(TRUE ("DO12")) -> ()  [unwired: 1 in, 1 out]
                      }
                      frame True {
                        w827 = FALSE ("DO8")
                        w830 = FALSE ("WasOff")
                        n258 = while {
                          shift-right: [w833] -> _
                          shift-left: _ -> [w832]
                          stop <- w834 stop-if-true
                          w837 = FALSE ("DO11")
                          n259 = shared-variable "RT CompactRIO Target\\Mod3\\DI13"() -> (w835:bool)  [unwired: 1 in, 1 out]
                          n260 = shared-variable "RT CompactRIO Target\\Mod3\\DI11"() -> (w836:bool)  [unwired: 1 in, 1 out]
                          n261 = shared-variable "RT CompactRIO Target\\Mod4\\DO11"(w837) -> ()  [unwired: 1 in, 1 out]
                          n262 = shared-variable "RT CompactRIO Target\\Mod4\\DO12"(w837) -> ()  [unwired: 1 in, 1 out]
                          n263 = Not(x=w832) -> (.not. x?=w833:bool)
                          n264 = shared-variable "RT CompactRIO Target\\Mod4\\DO0"(w832) -> ()  [unwired: 1 in, 1 out]
                          n265 = And(x=w836, y=w835) -> (x .and. y?=w834:bool)
                        }
                        n266 = shared-variable ".\\Untitled Library 1.lvlib\\WasRight"(TRUE ("WasOff")) -> ()  [unwired: 1 in, 1 out]
                        n267 = shared-variable ".\\Untitled Library 1.lvlib\\WasOff"(w830) -> ()  [unwired: 1 in, 1 out]
                        n268 = shared-variable "RT CompactRIO Target\\Mod4\\DO9"(w830) -> ()  [unwired: 1 in, 1 out]
                        n269 = shared-variable "RT CompactRIO Target\\Mod4\\DO0"(w827) -> ()  [unwired: 1 in, 1 out]
                        n270 = shared-variable "RT CompactRIO Target\\Mod4\\DO3"(w827) -> ()  [unwired: 1 in, 1 out]
                      }
                    }
                  }
                  frame True {
                    n271 = while {
                      stop <- w844 stop-if-true
                      w843 = FALSE ("DO8")
                      w848 = FALSE ("DO11")
                      n272 = shared-variable "RT CompactRIO Target\\Mod3\\DI11"() -> (w847:bool)  [unwired: 1 in, 1 out]
                      n273 = shared-variable "RT CompactRIO Target\\Mod3\\DI13"() -> (w846:bool)  [unwired: 1 in, 1 out]
                      n274 = shared-variable "RT CompactRIO Target\\Mod4\\DO11"(w848) -> ()  [unwired: 1 in, 1 out]
                      n275 = shared-variable "RT CompactRIO Target\\Mod4\\DO12"(w848) -> ()  [unwired: 1 in, 1 out]
                      n276 = And(x=w847, y=w846) -> (x .and. y?=w844:bool)
                      n277 = shared-variable "RT CompactRIO Target\\Mod4\\DO0"(w843) -> ()  [unwired: 1 in, 1 out]
                      n278 = shared-variable "RT CompactRIO Target\\Mod4\\DO4"(TRUE ("DO8")) -> ()  [unwired: 1 in, 1 out]
                      n279 = shared-variable "RT CompactRIO Target\\Mod4\\DO2"(w843) -> ()  [unwired: 1 in, 1 out]
                    }
                    n280 = shared-variable ".\\Untitled Library 1.lvlib\\WasEmergency"(FALSE ("WasEmergency")) -> ()  [unwired: 1 in, 1 out]
                    n281 = shared-variable "RT CompactRIO Target\\Mod4\\DO3"(FALSE ("DO3")) -> ()  [unwired: 1 in, 1 out]
                    n282 = shared-variable "RT CompactRIO Target\\Mod4\\DO9"(FALSE ("DO9")) -> ()  [unwired: 1 in, 1 out]
                  }
                }
              }
            }
          }
        }
        n283 = case shown="True" w611 {
          tunnel: [w889 w891] -> w608
          tunnel: [w889 w890] -> w610
          frame False {
            w889 = Control_1."Center" ("Enum")
          }
          frame True {
            n284 = flat-sequence {
              tunnel: [w996] -> w891
              tunnel: [w994] -> w890
              frame #0 {
                n285 = while {
                  shift-right: [w903] -> _
                  shift-left: FALSE ("DO8") -> [w904]
                  stop <- w897 stop-if-true
                  w902 = FALSE
                  n286 = shared-variable "RT CompactRIO Target\\Mod3\\DI1"() -> (w900:bool)  [unwired: 1 in, 1 out]
                  n287 = shared-variable "RT CompactRIO Target\\Mod3\\DI5"() -> (w893:bool)  [unwired: 1 in, 1 out]
                  n288 = shared-variable ".\\Untitled Library 1.lvlib\\WasOff"() -> (w896:bool)  [unwired: 1 in, 1 out]
                  n289 = case shown="True" w896 {
                    frame False {
                    }
                    frame True {
                      n290 = while {
                        shift-right: [w907] -> _
                        shift-left: FALSE -> [w909]
                        stop <- w908 stop-if-true
                        n291 = shared-variable "RT CompactRIO Target\\Mod3\\DI8"() -> (w908:bool)  [unwired: 1 in, 1 out]
                        n292 = Not(x=w909) -> (.not. x?=w907:bool)
                        n293 = shared-variable "RT CompactRIO Target\\Mod4\\DO0"(w907) -> ()  [unwired: 1 in, 1 out]
                      }
                    }
                  }
                  n294 = xnode "Edge Detect"("input 1"=w900) -> ("output"=w899:bool)  [unwired: 2 in, 1 out]
                  n295 = Not(x=w904) -> (.not. x?=w903:bool)
                  n296 = xnode "Edge Detect"("input 2"=w893) -> ("output"=w895:bool)  [unwired: 2 in, 1 out]
                  n297 = shared-variable "RT CompactRIO Target\\Mod4\\DO1"(w903) -> ()  [unwired: 1 in, 1 out]
                  n298 = case shown="True" w899 {
                    frame False {
                    }
                    frame True {
                      n299 = shared-variable "RT CompactRIO Target\\Untitled Library 1.lvlib\\System on"(FALSE ("System on")) -> ()  [unwired: 1 in, 1 out]
                      n300 = shared-variable ".\\Untitled Library 1.lvlib\\WasOff"(TRUE ("WasOff")) -> ()  [unwired: 1 in, 1 out]
                    }
                  }
                  n301 = case shown="True" w895 {
                    frame False {
                    }
                    frame True {
                      n302 = shared-variable ".\\Untitled Library 1.lvlib\\WasEmergency"(TRUE ("WasEmergency")) -> ()  [unwired: 1 in, 1 out]
                      n303 = shared-variable ".\\Untitled Library 1.lvlib\\System on"(FALSE ("System on")) -> ()  [unwired: 1 in, 1 out]
                    }
                  }
                  n304 = shared-variable "RT CompactRIO Target\\Mod4\\DO2"(FALSE ("DO2")) -> ()  [unwired: 1 in, 1 out]
                  n305 = shared-variable "RT CompactRIO Target\\Mod4\\DO10"(TRUE ("DO8")) -> ()  [unwired: 1 in, 1 out]
                  n306 = shared-variable "RT CompactRIO Target\\Mod3\\DI8"() -> (w894:bool)  [unwired: 1 in, 1 out]
                  n307 = shared-variable ".\\Untitled Library 1.lvlib\\WasEmergency"() -> (w898:bool)  [unwired: 1 in, 1 out]
                  n308 = shared-variable "RT CompactRIO Target\\Mod4\\DO11"(w902) -> ()  [unwired: 1 in, 1 out]
                  n309 = shared-variable "RT CompactRIO Target\\Mod4\\DO12"(w902) -> ()  [unwired: 1 in, 1 out]
                  n310 = Or(x=w898, y=w894) -> (x .or. y?=w897:bool)
                }
              }
              frame #1 {
                n311 = shared-variable ".\\Untitled Library 1.lvlib\\WasEmergency"() -> (w995:bool)  [unwired: 1 in, 1 out]
                n312 = case shown="False" w995 {
                  tunnel: [w998 Control_1."Emergency off" ("Enum")] -> w996
                  tunnel: [Control_1."Center" ("Enum") 0] -> w994
                  frame False {
                    n313 = shared-variable ".\\Untitled Library 1.lvlib\\WasOff"() -> (w999:bool)  [unwired: 1 in, 1 out]
                    n314 = case shown="False" w999 {
                      tunnel: [Control_1."Left" ("Enum") Control_1."System off" ("Enum")] -> w998
                      frame False {
                        n315 = shared-variable "RT CompactRIO Target\\Mod4\\DO10"(FALSE ("DO8")) -> ()  [unwired: 1 in, 1 out]
                        n316 = shared-variable "RT CompactRIO Target\\Mod4\\DO1"(TRUE ("DO3")) -> ()  [unwired: 1 in, 1 out]
                      }
                      frame True {
                        n317 = while {
                          shift-right: [w1008] -> _
                          shift-left: FALSE -> [w1007]
                          stop <- w1009 stop-if-true
                          n318 = Not(x=w1007) -> (.not. x?=w1008:bool)
                          n319 = shared-variable "RT CompactRIO Target\\Mod4\\DO0"(w1007) -> ()  [unwired: 1 in, 1 out]
                          n320 = shared-variable "RT CompactRIO Target\\Mod3\\DI8"() -> (w1009:bool)  [unwired: 1 in, 1 out]
                        }
                        n321 = shared-variable ".\\Untitled Library 1.lvlib\\WasOff"(FALSE ("WasOff")) -> ()  [unwired: 1 in, 1 out]
                        n322 = shared-variable "RT CompactRIO Target\\Mod4\\DO0"(FALSE ("DO2")) -> ()  [unwired: 1 in, 1 out]
                      }
                    }
                  }
                  frame True {
                    w1010 = FALSE ("WasEmergency")
                    n323 = shared-variable "RT CompactRIO Target\\Mod4\\DO1"(w1010) -> ()  [unwired: 1 in, 1 out]
                    n324 = shared-variable "RT CompactRIO Target\\Mod4\\DO4"(TRUE ("DO8")) -> ()  [unwired: 1 in, 1 out]
                    n325 = shared-variable ".\\Untitled Library 1.lvlib\\WasEmergency"(w1010) -> ()  [unwired: 1 in, 1 out]
                    n326 = shared-variable "RT CompactRIO Target\\Mod4\\DO10"(FALSE ("DO8")) -> ()  [unwired: 1 in, 1 out]
                    n327 = shared-variable "RT CompactRIO Target\\Mod4\\DO0"(FALSE ("DO2")) -> ()  [unwired: 1 in, 1 out]
                  }
                }
              }
            }
          }
        }
        n328 = case shown="True" w616 {
          tunnel: [Control_1."Center" ("Enum") Control_1."Emergency off" ("Enum")] -> w596
          frame False {
            n329 = shared-variable ".\\Untitled Library 1.lvlib\\WasCenter"(TRUE ("WasCenter")) -> ()  [unwired: 1 in, 1 out]
          }
          frame True {
            n330 = shared-variable "RT CompactRIO Target\\Untitled Library 1.lvlib\\System on"(FALSE ("System on")) -> ()  [unwired: 1 in, 1 out]
            n331 = shared-variable "RT CompactRIO Target\\Mod4\\DO0"(FALSE ("DO8")) -> ()  [unwired: 1 in, 1 out]
            n332 = shared-variable "RT CompactRIO Target\\Mod4\\DO2"(FALSE ("DO8")) -> ()  [unwired: 1 in, 1 out]
          }
        }
        n333 = Not(x=w614) -> (.not. x?=w613:bool)
        n334 = shared-variable "RT CompactRIO Target\\Untitled Library 1.lvlib\\CENTER"(w614) -> ()  [unwired: 1 in, 1 out]
        n335 = shared-variable "RT CompactRIO Target\\Untitled Library 1.lvlib\\EMERGENCY-OFF"(w613) -> ()  [unwired: 1 in, 1 out]
        n336 = shared-variable "RT CompactRIO Target\\Untitled Library 1.lvlib\\FAULT"(w613) -> ()  [unwired: 1 in, 1 out]
        n337 = shared-variable "RT CompactRIO Target\\Untitled Library 1.lvlib\\LEFT"(w613) -> ()  [unwired: 1 in, 1 out]
        n338 = shared-variable "RT CompactRIO Target\\Untitled Library 1.lvlib\\RIGHT"(w613) -> ()  [unwired: 1 in, 1 out]
        n339 = case shown="True" w617 {
          tunnel: [Control_1."Center" ("Enum") Control_1."System off" ("Enum")] -> w599
          frame False {
          }
          frame True {
            n340 = shared-variable ".\\Untitled Library 1.lvlib\\WasCenter"(TRUE ("WasCenter")) -> ()  [unwired: 1 in, 1 out]
            n341 = shared-variable "RT CompactRIO Target\\Untitled Library 1.lvlib\\System on"(FALSE ("System on")) -> ()  [unwired: 1 in, 1 out]
            n342 = shared-variable "RT CompactRIO Target\\Mod4\\DO0"(FALSE ("DO8")) -> ()  [unwired: 1 in, 1 out]
          }
        }
        n343 = Less?(x=w608, y=w610) -> (x < y?=w609:bool)
        n344 = Greater?(x=w603, y=w605) -> (0:w604:bool)
        n345 = Less?(x=w599, y=Control_1."Center") -> (x < y?=w600:bool)
        n346 = Greater?(x=w596, y=w594) -> (0:w597:bool)
        n347 = Select(t=w596, s=w597, f=w594) -> (s? t:f=w595:T1)
        n348 = Select(t=w599, s=w600, f=w595) -> (s? t:f=w598:T1)
        n349 = Select(t=w603, s=w604, f=w598) -> (s? t:f=w602:T1)
        n350 = Select(t=w608, s=w609, f=w602) -> (s? t:f=w592:T1)
      }
      frame "Left" {
        w1079 = FALSE ("SYSTEM-OFF")
        w1081 = TRUE ("RIGHT")
        w1060 = Control_1."Left" ("Enum")
        n351 = shared-variable "RT CompactRIO Target\\Mod3\\DI3"() -> (w1056:bool)  [unwired: 1 in, 1 out]
        n352 = xnode "Edge Detect"("input 1"=w1056) -> ("output"=w1087:bool)  [unwired: 2 in, 1 out]
        n353 = shared-variable "RT CompactRIO Target\\Untitled Library 1.lvlib\\System on"() -> (w1084:bool)  [unwired: 1 in, 1 out]
        n354 = shared-variable "RT CompactRIO Target\\Mod3\\DI4"() -> (w1058:bool)  [unwired: 1 in, 1 out]
        n355 = xnode "Edge Detect"("input 1"=w1058) -> ("output"=w1057:bool)  [unwired: 2 in, 1 out]
        n356 = shared-variable "RT CompactRIO Target\\Mod4\\DO0"(w1084) -> ()  [unwired: 1 in, 1 out]
        n357 = case shown="True" w1087 {
          tunnel: [w1359 w1361] -> w1076
          tunnel: [w1359 w1360] -> w1078
          frame False {
            w1359 = Control_1."Left" ("Enum")
          }
          frame True {
            n358 = flat-sequence {
              tunnel: [w1466] -> w1361
              tunnel: [w1464] -> w1360
              frame #0 {
                n359 = while {
                  shift-right: [w1373] -> _
                  shift-left: FALSE ("DO8") -> [w1374]
                  stop <- w1366 stop-if-true
                  n360 = shared-variable "RT CompactRIO Target\\Mod3\\DI5"() -> (w1364:bool)  [unwired: 1 in, 1 out]
                  n361 = shared-variable "RT CompactRIO Target\\Mod4\\DO1"(FALSE ("DO8")) -> ()  [unwired: 1 in, 1 out]
                  n362 = shared-variable "RT CompactRIO Target\\Mod4\\DO9"(TRUE ("DO8")) -> ()  [unwired: 1 in, 1 out]
                  n363 = shared-variable "RT CompactRIO Target\\Mod3\\DI1"() -> (w1370:bool)  [unwired: 1 in, 1 out]
                  n364 = xnode "Edge Detect"("input 2"=w1364) -> ("output"=w1363:bool)  [unwired: 2 in, 1 out]
                  n365 = xnode "Edge Detect"("input 1"=w1370) -> ("output"=w1369:bool)  [unwired: 2 in, 1 out]
                  n366 = case shown="True" w1363 {
                    frame False {
                    }
                    frame True {
                      n367 = shared-variable ".\\Untitled Library 1.lvlib\\WasEmergency"(TRUE ("WasEmergency")) -> ()  [unwired: 1 in, 1 out]
                      n368 = shared-variable ".\\Untitled Library 1.lvlib\\System on"(FALSE ("System on")) -> ()  [unwired: 1 in, 1 out]
                      n369 = shared-variable ".\\Untitled Library 1.lvlib\\WasCenter"(TRUE ("WasRight")) -> ()  [unwired: 1 in, 1 out]
                    }
                  }
                  n370 = case shown="True" w1369 {
                    frame False {
                    }
                    frame True {
                      n371 = shared-variable "RT CompactRIO Target\\Untitled Library 1.lvlib\\System on"(FALSE ("System on")) -> ()  [unwired: 1 in, 1 out]
                      n372 = shared-variable ".\\Untitled Library 1.lvlib\\WasOff"(TRUE ("WasOff")) -> ()  [unwired: 1 in, 1 out]
                    }
                  }
                  n373 = shared-variable ".\\Untitled Library 1.lvlib\\WasOff"() -> (w1365:bool)  [unwired: 1 in, 1 out]
                  n374 = case shown="True" w1365 {
                    frame False {
                    }
                    frame True {
                      (unwired) FALSE ("WasOff")
                      (unwired) FALSE ("DO8")
                      n375 = while {
                        shift-right: [w1376] -> _
                        shift-left: FALSE -> [w1378]
                        stop <- w1377 stop-if-true
                        n376 = shared-variable "RT CompactRIO Target\\Mod3\\DI9"() -> (w1377:bool)  [unwired: 1 in, 1 out]
                        n377 = Not(x=w1378) -> (.not. x?=w1376:bool)
                        n378 = shared-variable "RT CompactRIO Target\\Mod4\\DO0"(w1376) -> ()  [unwired: 1 in, 1 out]
                      }
                    }
                  }
                  n379 = Not(x=w1374) -> (.not. x?=w1373:bool)
                  n380 = shared-variable ".\\Untitled Library 1.lvlib\\WasEmergency"() -> (w1368:bool)  [unwired: 1 in, 1 out]
                  n381 = shared-variable "RT CompactRIO Target\\Mod4\\DO2"(w1373) -> ()  [unwired: 1 in, 1 out]
                  n382 = shared-variable "RT CompactRIO Target\\Mod3\\DI9"() -> (w1367:bool)  [unwired: 1 in, 1 out]
                  n383 = Or(x=w1367, y=w1368) -> (x .or. y?=w1366:bool)
                }
              }
              frame #1 {
                n384 = shared-variable ".\\Untitled Library 1.lvlib\\WasEmergency"() -> (w1465:bool)  [unwired: 1 in, 1 out]
                n385 = case shown="False" w1465 {
                  tunnel: [w1469 Control_1."Emergency off" ("Enum")] -> w1466
                  tunnel: [w1467 Control_1."Left" ("Enum")] -> w1464
                  frame False {
                    n386 = shared-variable ".\\Untitled Library 1.lvlib\\WasOff"() -> (w1468:bool)  [unwired: 1 in, 1 out]
                    n387 = case shown="False" w1468 {
                      tunnel: [Control_1."Center" ("Enum") Control_1."System off" ("Enum")] -> w1469
                      tunnel: [Control_1."Left" ("Enum") -1] -> w1467
                      frame False {
                        n388 = shared-variable "RT CompactRIO Target\\Mod4\\DO9"(FALSE ("DO8")) -> ()  [unwired: 1 in, 1 out]
                        n389 = shared-variable "RT CompactRIO Target\\Mod4\\DO2"(TRUE ("DO3")) -> ()  [unwired: 1 in, 1 out]
                      }
                      frame True {
                        n390 = shared-variable ".\\Untitled Library 1.lvlib\\WasOff"(FALSE ("WasOff")) -> ()  [unwired: 1 in, 1 out]
                        n391 = shared-variable "RT CompactRIO Target\\Mod4\\DO2"(TRUE ("DO3")) -> ()  [unwired: 1 in, 1 out]
                        n392 = shared-variable "RT CompactRIO Target\\Mod4\\DO9"(FALSE ("DO9")) -> ()  [unwired: 1 in, 1 out]
                        n393 = shared-variable ".\\Untitled Library 1.lvlib\\WasCenter"(TRUE ("WasRight")) -> ()  [unwired: 1 in, 1 out]
                      }
                    }
                  }
                  frame True {
                    w1480 = FALSE ("DO8")
                    n394 = shared-variable "RT CompactRIO Target\\Mod4\\DO2"(w1480) -> ()  [unwired: 1 in, 1 out]
                    n395 = shared-variable "RT CompactRIO Target\\Mod4\\DO9"(w1480) -> ()  [unwired: 1 in, 1 out]
                    n396 = shared-variable "RT CompactRIO Target\\Mod4\\DO0"(w1480) -> ()  [unwired: 1 in, 1 out]
                    n397 = shared-variable "RT CompactRIO Target\\Mod4\\DO4"(TRUE ("DO8")) -> ()  [unwired: 1 in, 1 out]
                    n398 = shared-variable ".\\Untitled Library 1.lvlib\\WasEmergency"(FALSE ("WasEmergency")) -> ()  [unwired: 1 in, 1 out]
                  }
                }
              }
            }
          }
        }
        n399 = case shown="True" w1057 {
          tunnel: [w1178 w1180] -> w1073
          tunnel: [w1178 w1179] -> w1075
          frame False {
            w1178 = Control_1."Left" ("Enum")
          }
          frame True {
            n400 = flat-sequence {
              tunnel: [w1288] -> w1180
              tunnel: [w1286] -> w1179
              frame #0 {
                n401 = while {
                  shift-right: [w1182] -> _
                  shift-left: FALSE ("DO8") -> [w1196]
                  stop <- w1184 stop-if-true
                  w1195 = TRUE ("DO8")
                  n402 = shared-variable "RT CompactRIO Target\\Mod3\\DI5"() -> (w1192:bool)  [unwired: 1 in, 1 out]
                  n403 = shared-variable ".\\Untitled Library 1.lvlib\\WasOff"() -> (w1189:bool)  [unwired: 1 in, 1 out]
                  n404 = shared-variable "RT CompactRIO Target\\Mod4\\DO9"(w1195) -> ()  [unwired: 1 in, 1 out]
                  n405 = shared-variable "RT CompactRIO Target\\Mod4\\DO11"(w1195) -> ()  [unwired: 1 in, 1 out]
                  n406 = xnode "Edge Detect"("input 2"=w1192) -> ("output"=w1193:bool)  [unwired: 2 in, 1 out]
                  n407 = shared-variable "RT CompactRIO Target\\Mod4\\DO12"(w1195) -> ()  [unwired: 1 in, 1 out]
                  n408 = case shown="True" w1189 {
                    frame False {
                    }
                    frame True {
                      n409 = while {
                        shift-right: [w1198] -> _
                        shift-left: FALSE -> [w1200]
                        stop <- w1199 stop-if-true
                        n410 = shared-variable "RT CompactRIO Target\\Mod3\\DI10"() -> (w1199:bool)  [unwired: 1 in, 1 out]
                        n411 = Not(x=w1200) -> (.not. x?=w1198:bool)
                        n412 = shared-variable "RT CompactRIO Target\\Mod4\\DO0"(w1198) -> ()  [unwired: 1 in, 1 out]
                      }
                    }
                  }
                  n413 = shared-variable "RT CompactRIO Target\\Mod4\\DO1"(FALSE ("DO8")) -> ()  [unwired: 1 in, 1 out]
                  n414 = Not(x=w1196) -> (.not. x?=w1182:bool)
                  n415 = case shown="True" w1193 {
                    frame False {
                    }
                    frame True {
                      n416 = shared-variable ".\\Untitled Library 1.lvlib\\System on"(FALSE ("System on")) -> ()  [unwired: 1 in, 1 out]
                      n417 = shared-variable ".\\Untitled Library 1.lvlib\\WasRight"(TRUE ("WasRight")) -> ()  [unwired: 1 in, 1 out]
                      n418 = shared-variable ".\\Untitled Library 1.lvlib\\WasEmergency"(TRUE ("WasEmergency")) -> ()  [unwired: 1 in, 1 out]
                    }
                  }
                  n419 = shared-variable "RT CompactRIO Target\\Mod3\\DI1"() -> (w1191:bool)  [unwired: 1 in, 1 out]
                  n420 = xnode "Edge Detect"("input 1"=w1191) -> ("output"=w1190:bool)  [unwired: 2 in, 1 out]
                  n421 = shared-variable "RT CompactRIO Target\\Mod3\\DI14"() -> (w1186:bool)  [unwired: 1 in, 1 out]
                  n422 = shared-variable "RT CompactRIO Target\\Mod4\\DO3"(w1182) -> ()  [unwired: 1 in, 1 out]
                  n423 = shared-variable "RT CompactRIO Target\\Mod3\\DI10"() -> (w1188:bool)  [unwired: 1 in, 1 out]
                  n424 = shared-variable "RT CompactRIO Target\\Mod3\\DI12"() -> (w1187:bool)  [unwired: 1 in, 1 out]
                  n425 = case shown="True" w1190 {
                    frame False {
                    }
                    frame True {
                      n426 = shared-variable "RT CompactRIO Target\\Untitled Library 1.lvlib\\System on"(FALSE ("System on")) -> ()  [unwired: 1 in, 1 out]
                      n427 = shared-variable ".\\Untitled Library 1.lvlib\\WasOff"(TRUE ("WasOff")) -> ()  [unwired: 1 in, 1 out]
                    }
                  }
                  n428 = Compound Arithmetic op=AND(w1188, w1187, w1186) -> (w1183:bool)
                  n429 = shared-variable ".\\Untitled Library 1.lvlib\\WasEmergency"() -> (w1185:bool)  [unwired: 1 in, 1 out]
                  n430 = Or(x=w1183, y=w1185) -> (x .or. y?=w1184:bool)
                }
              }
              frame #1 {
                n431 = shared-variable ".\\Untitled Library 1.lvlib\\WasEmergency"() -> (w1287:bool)  [unwired: 1 in, 1 out]
                n432 = case shown="False" w1287 {
                  tunnel: [w1291 Control_1."Emergency off" ("Enum")] -> w1288
                  tunnel: [w1289 Control_1."Left" ("Enum")] -> w1286
                  frame False {
                    n433 = shared-variable ".\\Untitled Library 1.lvlib\\WasOff"() -> (w1290:bool)  [unwired: 1 in, 1 out]
                    n434 = case shown="False" w1290 {
                      tunnel: [Control_1."Right" ("Enum") Control_1."System off" ("Enum")] -> w1291
                      tunnel: [Control_1."Left" ("Enum") -1] -> w1289
                      frame False {
                        n435 = shared-variable "RT CompactRIO Target\\Mod4\\DO9"(FALSE ("DO8")) -> ()  [unwired: 1 in, 1 out]
                        n436 = shared-variable "RT CompactRIO Target\\Mod4\\DO3"(TRUE ("DO12")) -> ()  [unwired: 1 in, 1 out]
                      }
                      frame True {
                        w1299 = FALSE ("WasOff")
                        n437 = while {
                          shift-right: [w1303] -> _
                          shift-left: FALSE -> [w1304]
                          stop <- w1305 stop-if-true
                          w1308 = FALSE ("DO11")
                          n438 = shared-variable "RT CompactRIO Target\\Mod3\\DI13"() -> (w1306:bool)  [unwired: 1 in, 1 out]
                          n439 = shared-variable "RT CompactRIO Target\\Mod3\\DI11"() -> (w1307:bool)  [unwired: 1 in, 1 out]
                          n440 = shared-variable "RT CompactRIO Target\\Mod4\\DO11"(w1308) -> ()  [unwired: 1 in, 1 out]
                          n441 = shared-variable "RT CompactRIO Target\\Mod4\\DO12"(w1308) -> ()  [unwired: 1 in, 1 out]
                          n442 = Not(x=w1304) -> (.not. x?=w1303:bool)
                          n443 = And(x=w1307, y=w1306) -> (x .and. y?=w1305:bool)
                          n444 = shared-variable "RT CompactRIO Target\\Mod4\\DO0"(w1303) -> ()  [unwired: 1 in, 1 out]
                        }
                        n445 = shared-variable ".\\Untitled Library 1.lvlib\\WasOff"(w1299) -> ()  [unwired: 1 in, 1 out]
                        n446 = shared-variable "RT CompactRIO Target\\Mod4\\DO3"(FALSE ("DO3")) -> ()  [unwired: 1 in, 1 out]
                        n447 = shared-variable "RT CompactRIO Target\\Mod4\\DO0"(FALSE ("DO8")) -> ()  [unwired: 1 in, 1 out]
                        n448 = shared-variable "RT CompactRIO Target\\Mod4\\DO9"(w1299) -> ()  [unwired: 1 in, 1 out]
                        n449 = shared-variable ".\\Untitled Library 1.lvlib\\WasRight"(TRUE ("WasOff")) -> ()  [unwired: 1 in, 1 out]
                      }
                    }
                  }
                  frame True {
                    n450 = while {
                      stop <- w1315 stop-if-true
                      w1314 = FALSE ("DO8")
                      w1318 = FALSE ("DO11")
                      n451 = shared-variable "RT CompactRIO Target\\Mod3\\DI13"() -> (w1316:bool)  [unwired: 1 in, 1 out]
                      n452 = shared-variable "RT CompactRIO Target\\Mod3\\DI11"() -> (w1317:bool)  [unwired: 1 in, 1 out]
                      n453 = shared-variable "RT CompactRIO Target\\Mod4\\DO11"(w1318) -> ()  [unwired: 1 in, 1 out]
                      n454 = shared-variable "RT CompactRIO Target\\Mod4\\DO12"(w1318) -> ()  [unwired: 1 in, 1 out]
                      n455 = And(x=w1317, y=w1316) -> (x .and. y?=w1315:bool)
                      n456 = shared-variable "RT CompactRIO Target\\Mod4\\DO4"(TRUE ("DO8")) -> ()  [unwired: 1 in, 1 out]
                      n457 = shared-variable "RT CompactRIO Target\\Mod4\\DO0"(w1314) -> ()  [unwired: 1 in, 1 out]
                      n458 = shared-variable "RT CompactRIO Target\\Mod4\\DO3"(w1314) -> ()  [unwired: 1 in, 1 out]
                    }
                    n459 = shared-variable ".\\Untitled Library 1.lvlib\\WasEmergency"(FALSE ("WasEmergency")) -> ()  [unwired: 1 in, 1 out]
                    n460 = shared-variable "RT CompactRIO Target\\Mod4\\DO9"(FALSE ("DO8")) -> ()  [unwired: 1 in, 1 out]
                  }
                }
              }
            }
          }
        }
        n461 = shared-variable "RT CompactRIO Target\\Mod3\\DI5"() -> (w1085:bool)  [unwired: 1 in, 1 out]
        n462 = shared-variable "RT CompactRIO Target\\Mod3\\DI1"() -> (w1086:bool)  [unwired: 1 in, 1 out]
        n463 = xnode "Edge Detect"("input 1"=w1086) -> ("output"=w1083:bool)  [unwired: 2 in, 1 out]
        n464 = xnode "Edge Detect"("input 2"=w1085) -> ("output"=w1082:bool)  [unwired: 2 in, 1 out]
        n465 = case shown="True" w1082 {
          tunnel: [Control_1."Left" ("Enum") Control_1."Emergency off" ("Enum")] -> w1062
          frame False {
          }
          frame True {
            n466 = shared-variable ".\\Untitled Library 1.lvlib\\WasEmergency"(TRUE ("WasEmergency")) -> ()  [unwired: 1 in, 1 out]
            n467 = shared-variable "RT CompactRIO Target\\Mod4\\DO0"(FALSE ("DO8")) -> ()  [unwired: 1 in, 1 out]
            n468 = shared-variable ".\\Untitled Library 1.lvlib\\System on"(FALSE ("System on")) -> ()  [unwired: 1 in, 1 out]
            n469 = shared-variable "RT CompactRIO Target\\Mod4\\DO1"(FALSE ("DO8")) -> ()  [unwired: 1 in, 1 out]
          }
        }
        n470 = case shown="True" w1083 {
          tunnel: [Control_1."Left" ("Enum") Control_1."System off" ("Enum")] -> w1065
          frame False {
          }
          frame True {
            n471 = shared-variable "RT CompactRIO Target\\Untitled Library 1.lvlib\\System on"(FALSE ("System on")) -> ()  [unwired: 1 in, 1 out]
            n472 = shared-variable ".\\Untitled Library 1.lvlib\\WasOff"(TRUE ("WasOff")) -> ()  [unwired: 1 in, 1 out]
          }
        }
        n473 = shared-variable "RT CompactRIO Target\\Untitled Library 1.lvlib\\SYSTEM-OFF"(w1079) -> ()  [unwired: 1 in, 1 out]
        n474 = shared-variable "RT CompactRIO Target\\Untitled Library 1.lvlib\\SYSTEM-ON"(w1079) -> ()  [unwired: 1 in, 1 out]
        n475 = Not(x=w1081) -> (.not. x?=w1080:bool)
        n476 = shared-variable "RT CompactRIO Target\\Untitled Library 1.lvlib\\CENTER"(w1080) -> ()  [unwired: 1 in, 1 out]
        n477 = shared-variable "RT CompactRIO Target\\Untitled Library 1.lvlib\\EMERGENCY-OFF"(w1080) -> ()  [unwired: 1 in, 1 out]
        n478 = shared-variable "RT CompactRIO Target\\Untitled Library 1.lvlib\\FAULT"(w1080) -> ()  [unwired: 1 in, 1 out]
        n479 = shared-variable "RT CompactRIO Target\\Untitled Library 1.lvlib\\LEFT"(w1081) -> ()  [unwired: 1 in, 1 out]
        n480 = shared-variable "RT CompactRIO Target\\Untitled Library 1.lvlib\\RIGHT"(w1080) -> ()  [unwired: 1 in, 1 out]
        n481 = shared-variable "RT CompactRIO Target\\Mod3\\DI11"() -> (w1070:bool)  [unwired: 1 in, 1 out]
        n482 = shared-variable "RT CompactRIO Target\\Mod3\\DI13"() -> (w1069:bool)  [unwired: 1 in, 1 out]
        n483 = shared-variable "RT CompactRIO Target\\Mod3\\DI8"() -> (w1071:bool)  [unwired: 1 in, 1 out]
        n484 = Compound Arithmetic op=AND(w1071, w1070, w1069) -> (w1068:bool)
        n485 = Less?(x=w1065, y=Control_1."Left" ("Enum")) -> (x < y?=w1066:bool)
        n486 = Greater?(x=w1062, y=w1060) -> (0:w1063:bool)
        n487 = shared-variable "RT CompactRIO Target\\Mod4\\DO1"(w1068) -> ()  [unwired: 1 in, 1 out]
        n488 = Greater?(x=w1073, y=w1075) -> (0:w1074:bool)
        n489 = Greater?(x=w1076, y=w1078) -> (0:w1077:bool)
        n490 = Select(t=w1062, s=w1063, f=w1060) -> (s? t:f=w1061:T1)
        n491 = Select(t=w1065, s=w1066, f=w1061) -> (s? t:f=w1064:T1)
        n492 = Select(t=w1073, s=w1074, f=w1064) -> (s? t:f=w1072:T1)
        n493 = Select(t=w1076, s=w1077, f=w1072) -> (s? t:f=w1059:T1)
      }
      frame "System off", Default {
        w1525 = FALSE ("SYSTEM-ON")
        n494 = shared-variable "RT CompactRIO Target\\Mod3\\DI0"() -> (w1534:bool)  [unwired: 1 in, 1 out]
        n495 = shared-variable "RT CompactRIO Target\\Mod3\\DI11"() -> (w1529:bool)  [unwired: 1 in, 1 out]
        n496 = shared-variable "RT CompactRIO Target\\Mod3\\DI13"() -> (w1528:bool)  [unwired: 1 in, 1 out]
        n497 = shared-variable "RT CompactRIO Target\\Mod3\\DI8"() -> (w1530:bool)  [unwired: 1 in, 1 out]
        n498 = xnode "Edge Detect"("input 1"=w1534) -> ("output"=w1533:bool)  [unwired: 2 in, 1 out]
        n499 = Compound Arithmetic op=AND(w1530, w1529, w1528) -> (w1527:bool)
        n500 = shared-variable "RT CompactRIO Target\\Untitled Library 1.lvlib\\System on"() -> (w1531:bool)  [unwired: 1 in, 1 out]
        n501 = case shown="True" w1533 {
          selector: w1533 -> [_ w1579]
          tunnel: [_ Control_1."System on" ("Enum")] -> w1532
          frame False {
          }
          frame True {
            n502 = shared-variable ".\\Untitled Library 1.lvlib\\WasCenter"() -> (w1577:bool)  [unwired: 1 in, 1 out]
            n503 = shared-variable ".\\Untitled Library 1.lvlib\\WasRight"() -> (w1576:bool)  [unwired: 1 in, 1 out]
            n504 = shared-variable "RT CompactRIO Target\\Untitled Library 1.lvlib\\System on"(w1579) -> ()  [unwired: 1 in, 1 out]
            n505 = Or(x=w1577, y=w1576) -> (x .or. y?=w1575:bool)
            n506 = case shown="True" w1575 {
              frame False {
              }
              frame True {
                n507 = flat-sequence {
                  frame #0 {
                    n508 = while {
                      stop <- w1581 stop-if-true
                      w1580 = TRUE ("DO10")
                      n509 = shared-variable "RT CompactRIO Target\\Mod3\\DI8"() -> (w1581:bool)  [unwired: 1 in, 1 out]
                      n510 = shared-variable "RT CompactRIO Target\\Mod4\\DO10"(w1580) -> ()  [unwired: 1 in, 1 out]
                      n511 = shared-variable "RT CompactRIO Target\\Mod4\\DO0"(w1580) -> ()  [unwired: 1 in, 1 out]
                    }
                  }
                  frame #1 {
                    n512 = shared-variable ".\\Untitled Library 1.lvlib\\WasCenter"(FALSE ("WasCenter")) -> ()  [unwired: 1 in, 1 out]
                    n513 = shared-variable "RT CompactRIO Target\\Mod4\\DO10"(FALSE ("DO10")) -> ()  [unwired: 1 in, 1 out]
                    n514 = shared-variable "RT CompactRIO Target\\Mod4\\DO2"(FALSE ("DO10")) -> ()  [unwired: 1 in, 1 out]
                    n515 = shared-variable ".\\Untitled Library 1.lvlib\\WasRight"(FALSE ("WasCenter")) -> ()  [unwired: 1 in, 1 out]
                  }
                }
              }
            }
          }
        }
        n516 = shared-variable "RT CompactRIO Target\\Mod4\\DO0"(w1531) -> ()  [unwired: 1 in, 1 out]
        n517 = shared-variable "RT CompactRIO Target\\Mod4\\DO1"(w1527) -> ()  [unwired: 1 in, 1 out]
        n518 = shared-variable "RT CompactRIO Target\\Untitled Library 1.lvlib\\SYSTEM-OFF"(TRUE ("SYSTEM-OFF")) -> ()  [unwired: 1 in, 1 out]
        n519 = shared-variable "RT CompactRIO Target\\Untitled Library 1.lvlib\\SYSTEM-ON"(w1525) -> ()  [unwired: 1 in, 1 out]
        n520 = shared-variable "RT CompactRIO Target\\Untitled Library 1.lvlib\\CENTER"(w1525) -> ()  [unwired: 1 in, 1 out]
        n521 = shared-variable "RT CompactRIO Target\\Untitled Library 1.lvlib\\EMERGENCY-OFF"(w1525) -> ()  [unwired: 1 in, 1 out]
        n522 = shared-variable "RT CompactRIO Target\\Untitled Library 1.lvlib\\FAULT"(w1525) -> ()  [unwired: 1 in, 1 out]
        n523 = shared-variable "RT CompactRIO Target\\Untitled Library 1.lvlib\\LEFT"(w1525) -> ()  [unwired: 1 in, 1 out]
        n524 = shared-variable "RT CompactRIO Target\\Untitled Library 1.lvlib\\RIGHT"(w1525) -> ()  [unwired: 1 in, 1 out]
      }
      frame "System on" {
        w1588 = FALSE ("SYSTEM-ON")
        n525 = shared-variable "RT CompactRIO Target\\Mod3\\DI1"() -> (w1587:bool)  [unwired: 1 in, 1 out]
        n526 = shared-variable "RT CompactRIO Target\\Mod3\\DI11"() -> (w1592:bool)  [unwired: 1 in, 1 out]
        n527 = shared-variable "RT CompactRIO Target\\Mod3\\DI13"() -> (w1591:bool)  [unwired: 1 in, 1 out]
        n528 = shared-variable "RT CompactRIO Target\\Mod3\\DI8"() -> (w1593:bool)  [unwired: 1 in, 1 out]
        n529 = Compound Arithmetic op=AND(w1593, w1592, w1591) -> (w1590:bool)
        n530 = xnode "Edge Detect"("input 1"=w1587) -> ("output"=w1586:bool)  [unwired: 2 in, 1 out]
        n531 = shared-variable "RT CompactRIO Target\\Untitled Library 1.lvlib\\System on"() -> (w1595:bool)  [unwired: 1 in, 1 out]
        n532 = shared-variable "RT CompactRIO Target\\Mod4\\DO1"(w1590) -> ()  [unwired: 1 in, 1 out]
        n533 = case shown="True" w1586 {
          selector: w1586 -> [_ w1639]
          tunnel: [Control_1."Left" ("Enum") Control_1."System off" ("Enum")] -> w1594
          frame False {
          }
          frame True {
            n534 = Not(x=w1639) -> (.not. x?=w1638:bool)
            n535 = shared-variable "RT CompactRIO Target\\Untitled Library 1.lvlib\\System on"(w1638) -> ()  [unwired: 1 in, 1 out]
          }
        }
        n536 = shared-variable "RT CompactRIO Target\\Mod4\\DO0"(w1595) -> ()  [unwired: 1 in, 1 out]
        n537 = shared-variable "RT CompactRIO Target\\Untitled Library 1.lvlib\\SYSTEM-OFF"(w1588) -> ()  [unwired: 1 in, 1 out]
        n538 = shared-variable "RT CompactRIO Target\\Untitled Library 1.lvlib\\SYSTEM-ON"(TRUE ("SYSTEM-OFF")) -> ()  [unwired: 1 in, 1 out]
        n539 = shared-variable "RT CompactRIO Target\\Untitled Library 1.lvlib\\CENTER"(w1588) -> ()  [unwired: 1 in, 1 out]
        n540 = shared-variable "RT CompactRIO Target\\Untitled Library 1.lvlib\\EMERGENCY-OFF"(w1588) -> ()  [unwired: 1 in, 1 out]
        n541 = shared-variable "RT CompactRIO Target\\Untitled Library 1.lvlib\\FAULT"(w1588) -> ()  [unwired: 1 in, 1 out]
        n542 = shared-variable "RT CompactRIO Target\\Untitled Library 1.lvlib\\LEFT"(w1588) -> ()  [unwired: 1 in, 1 out]
        n543 = shared-variable "RT CompactRIO Target\\Untitled Library 1.lvlib\\RIGHT"(w1588) -> ()  [unwired: 1 in, 1 out]
      }
    }
  }
